vi "VHist - Fit STR history to new timestamps.vi"(4 "merge data (T)":bool=TRUE, 6 "empty for absent (T)":bool=TRUE, 7 "new time stamps":dbl[](array[numeric]) format="%<%H:%M:%S%2u\n%d/%m/%Y>T", 8 "error in":errorcluster, 9 "time condition":cluster{"From":dbl, "To":dbl, "step, sec":dbl} {"step, sec" format="%.2f"; "To" format="%<%H:%M:%S%2u\n%d/%m/%Y>T"; "From" format="%<%H:%M:%S%2u\n%d/%m/%Y>T"}, 10 "history data":string[](array[string]), 11 "time stamps":dbl[](array[numeric]) format="%<%H:%M:%S%3u\n%d/%m/%Y>T") -> (0 "error out":errorcluster, 2 "history data out":string[](array[string]), 3 "time stamps out":dbl[](array[numeric]) format="%<%H:%M:%S%2u\n%d/%m/%Y>T")   [LabVIEW 2021]
doc: "The VI looks over String history and determines history values at the new time stamps specified. New time stamps can be specified either in <b>new time stamps</b> array or <b>time conditions</b> cluster defining initial and final timestamps, and time step. By default, VI replaces absent values with an empty string and merges values located between adjacent new time stamps. Either of these features can be suppressed.\n\n::: CalcExpress Toolkit :::\nCopyright (c) 2000-2026 Konstantin Shifershteyn. All rights reserved."
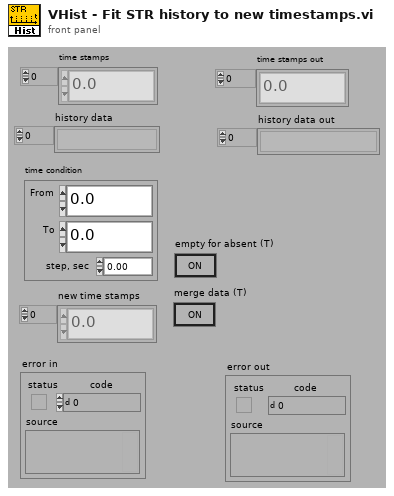
[diagram p1: front panel]
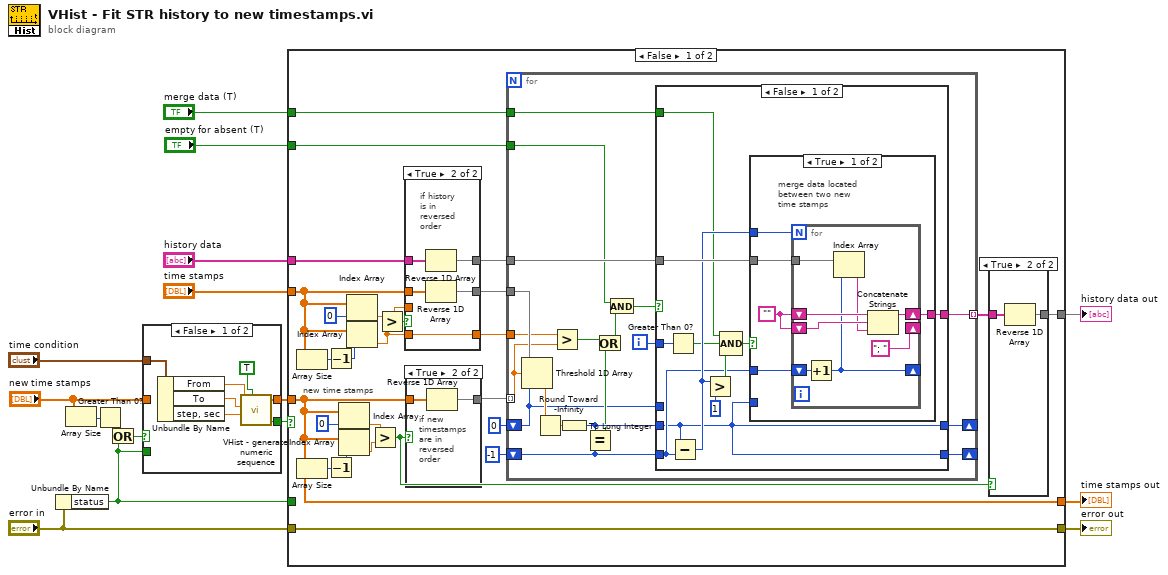
[diagram p0: block diagram]
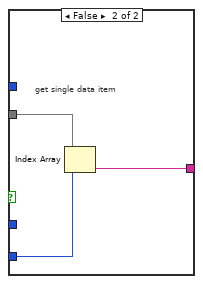
[diagram p3: hidden frame]
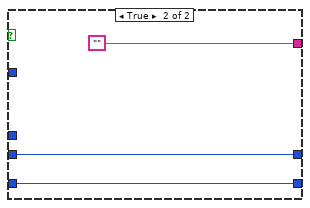
[diagram p4: hidden frame]
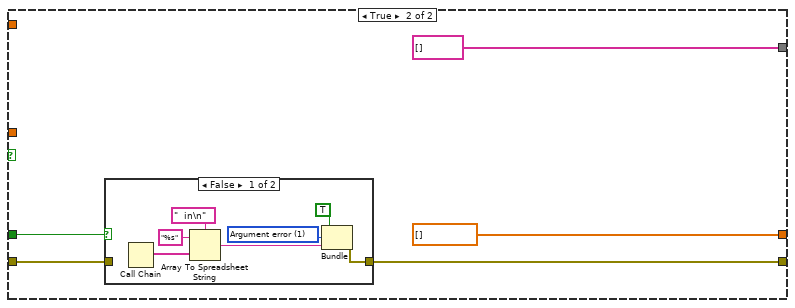
[diagram p8: hidden frame]
diagram:
  n1 = Unbundle By Name("error in") -> ("status"=w3:bool)
  n2 = Array Size(array="new time stamps") -> (size(s)=w12:i32)
  n3 = Greater Than 0?(x=w12) -> (x > 0?=w11:bool)
  n4 = Or(x=w11, y=w3) -> (x .or. y?=w4:bool)
  n5 = case shown="False" w4 {
    tunnel: [w22 w25] -> w8
    tunnel: "new time stamps" -> [_ w25]
    tunnel: "time condition" -> [w23 _]
    tunnel: [w17 w24] -> w7
    tunnel: w3 -> [_ w24]
    frame False {
      n6 = Unbundle By Name(w23) -> ("From"=w19:dbl, "To"=w20:dbl, "step, sec"=w21:dbl)
      n7 = call "VHist - generate numeric sequence.vi"("inclusive (T)"=TRUE, "step"=w21, "final value"=w20, "initial value"=w19) -> ("error"=w17:bool, "array out"=w22:dbl[])  [unwired: 4 in]
    }
    frame True {
    }
  }
  n8 = case shown="False" w7 {
    tunnel: "error in" -> [w51 w118]
    tunnel: w3 -> [_ w119]
    tunnel: [w51 w117] -> w15
    tunnel: [w38 dbl[] []] -> w14
    tunnel: [w39 string[] []] -> w13
    tunnel: w8 -> [w38 _]
    tunnel: "time stamps" -> [w47 _]
    tunnel: "history data" -> [w46 _]
    tunnel: "merge data (T)" -> [w27 _]
    tunnel: "empty for absent (T)" -> [w26 _]
    frame False {
      # "new time stamps"
      n9 = Array Size(array=w47) -> (size(s)=w49:i32)
      n10 = Array Size(array=w38) -> (size(s)=w41:i32)
      n11 = Decrement(x=w49) -> (x-1=w29:i32)
      n12 = Decrement(x=w41) -> (x-1=w42:i32)
      n13 = Index Array(array=w38, index=0) -> (element=w44:dbl)
      n14 = Index Array(array=w38, index=w42) -> (element=w45:dbl)
      n15 = Index Array(array=w47, index=0) -> (element=w30:dbl)
      n16 = Index Array(array=w47, index=w29) -> (element=w32:dbl)
      n17 = Greater?(x=w44, y=w45) -> (0:w40:bool)
      n18 = Greater?(x=w30, y=w32) -> (0:w50:bool)
      n19 = case shown="True" w50 {
        tunnel: w47 -> [w109 w114]
        tunnel: [w109 w113] -> w35
        tunnel: w46 -> [w108 w112]
        tunnel: [w108 w111] -> w34
        tunnel: [w107 w110] -> w31
        tunnel: w32 -> [_ w110]
        tunnel: w30 -> [w107 _]
        frame False {
        }
        frame True {
          # "if history\nis in\nreversed\norder"
          n20 = Reverse 1D Array(array=w112) -> (reversed array=w111:string[])
          n21 = Reverse 1D Array(array=w114) -> (reversed array=w113:dbl[])
        }
      }
      n22 = case shown="True" w40 {
        tunnel: w38 -> [w104 w106]
        tunnel: [w104 w105] -> w36
        frame False {
        }
        frame True {
          # "if new\ntimestamps\nare in\nreversed\norder"
          n23 = Reverse 1D Array(array=w106) -> (reversed array=w105:dbl[])
        }
      }
      n24 = for {
        tunnel: w34 -> [w70]
        tunnel: w35 -> [w69]
        tunnel: w36 -> [w63] mode=indexing
        tunnel: [w68] -> w33 mode=indexing
        shift-right: [w61] -> _
        shift-left: 0 -> [w56]
        shift-right: [w60] -> _
        shift-left: -1 -> [w57]
        tunnel: w31 -> [w64]
        tunnel: w27 -> [w53]
        tunnel: w26 -> [w52]
        i -> [w54]
        n25 = Threshold 1D Array(1:w56, 2:w63, 3:w69) -> (0:w66:dbl)
        n26 = Round Toward -Infinity(1:w66) -> (0:w65:dbl)
        n27 = Greater?(x=w64, y=w63) -> (0:w55:bool)
        n28 = To Long Integer(number=w65) -> (32bit integer=w62:i32)
        n29 = Equal?(x=w62, y=w57) -> (x = y?=w59:bool)
        n30 = Or(x=w55, y=w59) -> (x .or. y?=w58:bool)
        n31 = And(x=w52, y=w58) -> (x .and. y?=w67:bool)
        n32 = case shown="False" w67 {
          tunnel: w70 -> [w80 _]
          tunnel: [w81 ""] -> w68
          tunnel: w62 -> [w72 w99]
          tunnel: [w72 w99] -> w61
          tunnel: w57 -> [w73 w98]
          tunnel: [w72 w98] -> w60
          tunnel: w56 -> [_ _]
          tunnel: w54 -> [w75 _]
          tunnel: w53 -> [w71 _]
          frame False {
            n33 = Greater Than 0?(x=w75) -> (x > 0?=w76:bool)
            n34 = Subtract(x=w72, y=w73) -> (x-y=w77:i32)
            n35 = Greater?(x=w77, y=1 ("x")) -> (0:w74:bool)
            n36 = Compound Arithmetic op=AND(w71, w76, w74) -> (w79:bool)
            n37 = case shown="True" w79 {
              tunnel: [w85 w97] -> w81
              tunnel: w80 -> [w82 w96]
              tunnel: w73 -> [w83 _]
              tunnel: w72 -> [_ w95]
              tunnel: w77 -> [w84 _]
              frame True {
                w86 = ""
                # "merge data located\nbetween two new\ntime stamps"
                n38 = for {
                  N: w84 -> [_]
                  shift-right: [w92] -> w85
                  shift-left: w86 -> [w93]
                  shift-right: ["; "] -> _
                  shift-left: w86 -> [w91]
                  shift-right: [w88] -> _
                  shift-left: w83 -> [w89]
                  tunnel: w82 -> [w87]
                  n39 = Increment(x=w89) -> (x+1=w88:i32)
                  n40 = Index Array(array=w87, index=w88) -> (element=w90:string)
                  n41 = Concatenate Strings(w93, w91, w90) -> (w92:string)
                }
              }
              frame False {
                # "get single data item"
                n42 = Index Array(array=w96, index=w95) -> (element=w97:string)
              }
            }
          }
          frame True {
          }
        }
      }
      n43 = case shown="True" w40 {
        tunnel: w33 -> [w101 w103]
        tunnel: [w101 w102] -> w39
        frame False {
        }
        frame True {
          n44 = Reverse 1D Array(array=w103) -> (reversed array=w102:string[])
        }
      }
    }
    frame True {
      n45 = case shown="False" w119 {
        tunnel: [w126 w127] -> w117
        tunnel: w118 -> [_ w127]
        frame False {
          w124 = 1 items=["No error", "Argument error", "Memory is full", "Out of zone", "End of file", "File already open", "Generic file I/O error", "File not found", "File permission error", "Disk is full", "Duplicate path", "Too many files open", "System feature not enabled", "Resource file not found", "Cannot add resource", "Resource not found", "Image not found", "Image memory error", "Pen does not exist", "Config type invalid", "Config token not found", "Config parse error", "Config memory error", "Bad external code format", "Bad external code offset", "External code not present", "Null window", "Destroy window error", "Null menu", "Print aborted", "Bad print record", "Print driver error", "Windows error during printing", "Memory error during printing", "Print dialog error", "Generic print error", "Invalid device refnum", "Device not found", "Device parameter error", "Device unit error", "Cannot open device", "Device call aborted", "Generic error", "Cancelled by user", "Object ID too low", "Object ID too high", "Object not in heap", "Unknown heap", "Unknown object (invalid DefProc)", "Unknown object (DefProc not in table)", "Message out of range", "Invalid (null) method", "Unknown message", "Manager call not supported", "Bad address", "Network operation in progress", "Network operation timed out", "Connection is busy", "Network attribute not supported", "Network error", "Address in use", "System out of memory", "Connection aborted", "Connection refused", "Not connected", "Already connected", "Connection closed", "Initialization error (interapplication manager)", "Bad occurrence", "Wait on unbound occurrence handler", "Occurrence queue overflow", "Datalog type conflict", "Unused", "Unrecognized type (interapplication manager)", "Memory corrupt", "Failed to make temporary DLL", "Old CIN version", "Drag socket not found", "Failed to load drop-object", "Failed to register OLE object", "Failed to release OLE object", "Format specifier type mismatch", "Unknown format specifier", "Too few format specifiers", "Too many format specifiers", "Scan failed", "Newer CIN version", "Error converting to variant", "Runtime menu error", "Password tampered", "Variant attribute not found", "Incompatible variant data type", "Event data is not available", "Event Store is not present", "Occurrence is not found", "Event Queue is not created", "Event info is not available", "Refnum passed is NULL", "Error retrieving Class GUID", "Error retrieving CoClass GUID", "Error retrieving TypeLib GUID.", "Bad built application magic bytes.", "Specific driver is different from the specific driver associated with the Logical Name.", "There is no session opened to the class driver.", "Max Error", "MAX - Error with config objects", "MAX - Error loading configuration", "MAX - Group not supported"]
          n46 = Call Chain() -> (call chain=w123:string[])
          n47 = Array To Spreadsheet String(delimiter (Tab)="  in\n", array=w123, 3:"%s" ("format string")) -> (spreadsheet string=w120:string)
          n48 = Bundle(TRUE, w124, "spreadsheet string"=w120) -> (w126:cluster{bool, i32, "spreadsheet string":string})  [unwired: 1 in]
        }
        frame True {
        }
      }
    }
  }
  "error out" <- w15
  "history data out" <- w13
  "time stamps out" <- w14
